vi "Create Boolean Input Channels.vi"(8 "error in (no error)":errorcluster, 11 "Modbus in":refnum<class "Modbus.lvclass">) -> (0 "error out":errorcluster, 1 "Channels to remove":string[](array[string]), 3 "Modbus out":refnum<class "Modbus.lvclass">)   [LabVIEW 2026, in "Modbus.lvlib" / "Modbus.lvclass"]
uses:
  Modbus.lvclass
  C:/Program Files/National Instruments/LabVIEW 2026/vi.lib/FlexLogger/SDK/PluginSDK.lvlibp/PEFClasses/SDK/Plugin/Plugin.lvclass
  Modbus.lvclass/Modbus.ctl
  Globals/Modbus Strings.vi
  <vilib>/FlexLogger/SDK/PluginSDK.lvlibp/PEFClasses/SDK/Plugin/ParameterAccess/Read I32.vi
  <vilib>/FlexLogger/SDK/PluginSDK.lvlibp/PEFClasses/SDK/Plugin/Plugin.lvclass
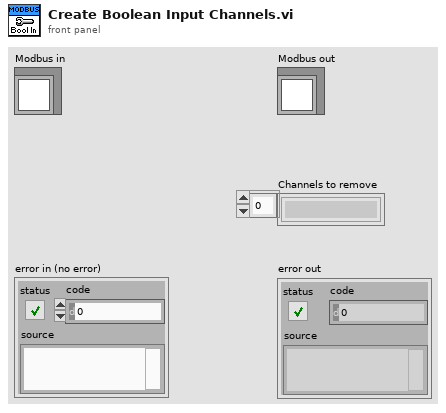
[diagram p1: front panel]
types:
  T1 = typedef "Modbus.lvlib/Modbus.lvclass/Boolean Data.ctl" = cluster{"Channel UID":string, "Valid?":bool, "Table":T2, "Address":i32}
  T2 = typedef "Modbus.lvlib/Modbus.lvclass/Modbus Table.ctl" = enum16{"Discrete Inputs", "Coils", "Input Registers", "Holding Registers"}
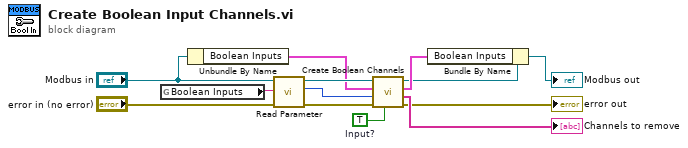
[diagram p0: block diagram]
diagram:
  w4 = TRUE  # Input?
  n1 = global read "Modbus Strings.vi" "Boolean Inputs"() -> (w10:string)
  n2 = Unbundle By Name("Modbus in") -> ("Boolean Inputs"=w6:T1[])
  n3 = call-poly <vilib>:"Read Parameter.vi"("error in (no error)"="error in (no error)", "Name"=w10, "Plugin in"="Modbus in") -> ("error out"=w8:errorcluster, "Value"=w7:i32, "Plugin out"=w9:refnum<class "Modbus.lvclass">)  [unwired: 5 in, 1 out]
  n4 = call "Create Boolean Channels.vi"("Input?"=w4, "error in (no error)"=w8, "New Number of Channels"=w7, "Boolean Channels in"=w6, "Modbus in"=w9) -> ("error out"=→"error out":errorcluster, "Channels to remove"=→"Channels to remove":string[], "Boolean channels out"=w5:T1[], "Modbus out"=w2:refnum<class "Modbus.lvclass">)  [unwired: 3 in]
  n5 = Bundle By Name(cluster=w2, "Boolean Inputs"=w5) -> (→"Modbus out":refnum<class "Modbus.lvclass">)
